vi "Guardian Died Recheck.vi"(8 "error in (no error)":errorcluster, 10 "ID":string, 11 "Guardian in":refnum<class "Guardian.lvclass">) -> (0 "error out":errorcluster, 3 "Guardian out":refnum<class "Guardian.lvclass">)   [LabVIEW 2020, in "TALOS.lvlib" / "Guardian.lvlib" / "Guardian.lvclass"]
doc: "This VI gets scheduled to be run whenever a Guardian is found to be not updating its Guardian_Health ASV: if the Guardian is found alive, nothing is done, while if it is really found dead, ABORT is raised."
uses:
  Guardian.lvclass
  Guardian.lvclass/Guardian.ctl
  TALOS.lvlib
  Classes/Distributed uService Map/Distributed uService Map.lvclass
  d99af1e7-28a1-4e92-bcbf-3239d693d740.vi
  Ancestor/Ancestor/Ancestor.lvclass
  C:/LabVIEW Code/TALOS/talos/Ancestor/Ancestor/Ancestor.lvclass
  C:/LabVIEW Code/TALOS/builds/Actor Framework PPL/Actor Framework.lvlibp/1abvi3w/vi.lib/ActorFramework/Actor/Actor.lvclass
  C:/LabVIEW Code/TALOS/talos/Guardian/Guardian/Guardian.lvclass
  Classes/Guardian List/Guardian List.lvclass
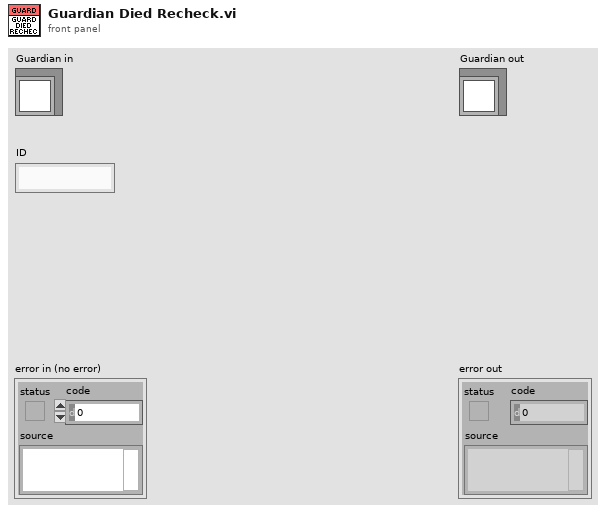
[diagram p1: front panel]
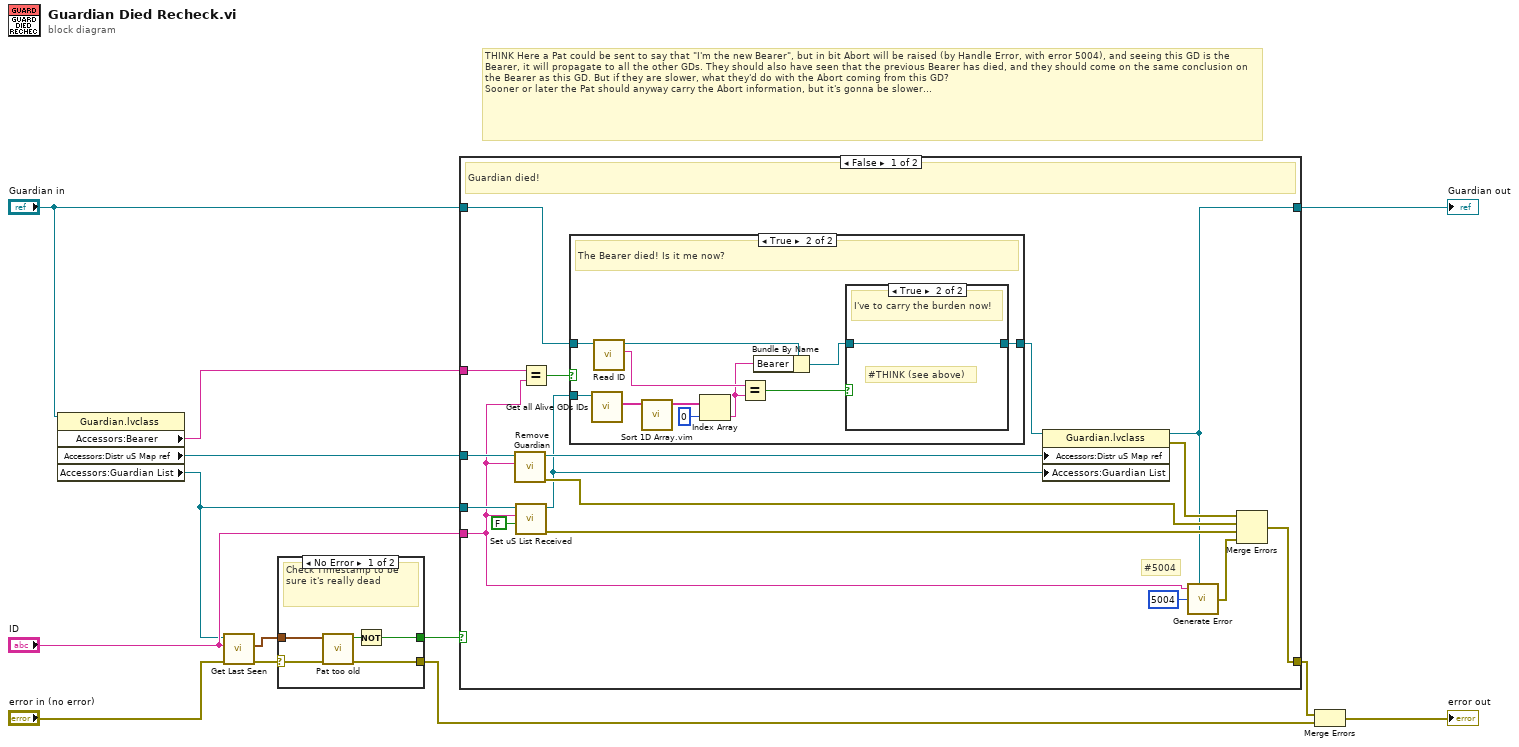
[diagram p0: block diagram]
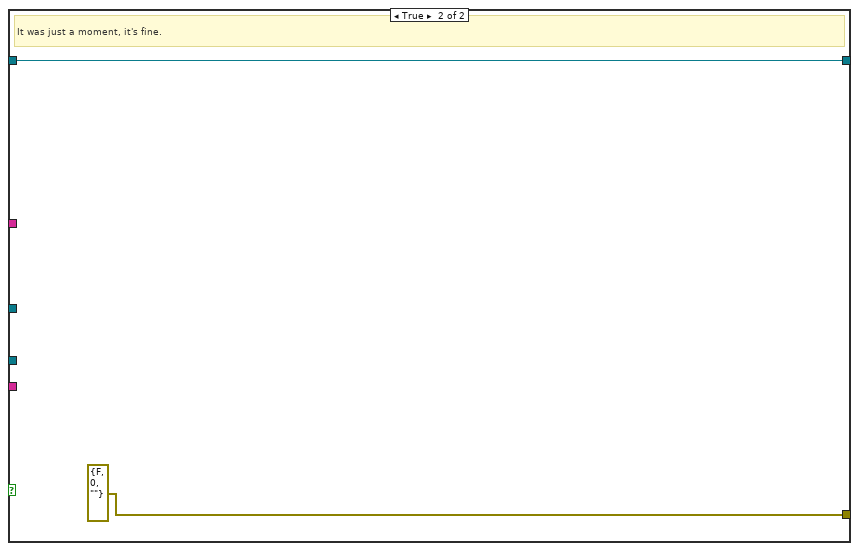
[diagram p4: hidden frame]
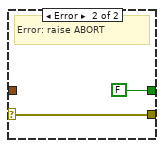
[diagram p5: hidden frame]
diagram:
  # "THINK Here a Pat could be sent to say that \"I'm the new Bearer\", but in bit Abort will be raised (by Handle Error, with error 5004), and seeing this GD is the Bearer, it will propagate to all the other GDs. They should also have seen that the previous Bearer has died, and they should come on the same conclusion on the Bearer as this GD. But if they are slower, what they'd do with the Abort coming from this GD? \nSooner or later the Pat should anyway carry the Abort information, but it's gonna be slower..."
  n1 = property class="Guardian.lvclass"(reference="Guardian in") -> ("Accessors:Bearer"=w1:string, "Accessors:Distr uS Map ref"=w2:refnum<data-value>, "Accessors:Guardian List"=w3:refnum<class "Guardian List.lvclass">)  [unwired: 1 in, 2 out]
  n2 = call-dynamic "Get Last Seen.vi"("error in (no error)"="error in (no error)", "ID"="ID", "Guardian List in"=w3) -> ("error out"=w8:errorcluster, "Last Poke"=w9:timestamp)  [unwired: 6 in, 1 out]
  n3 = case shown="No Error" w8 {
    selector: w8 -> [w15 w19]
    tunnel: w9 -> [w18 _]
    tunnel: [w16 FALSE] -> w11
    tunnel: [w14 w19] -> w7
    frame No Error {
      # "Check Timestamp to be sure it's really dead"
      n4 = call "Pat too old.vi"("error in (no error)"=w15, "Last Seen"=w18) -> ("error out"=w14:errorcluster, "Too old?"=w17:bool)  [unwired: 8 in]
      n5 = Not(x=w17) -> (.not. x?=w16:bool)
    }
    frame Error {
      # "Error: raise ABORT"
    }
  }
  n6 = case shown="False" w11 {
    tunnel: [w34 errorcluster {"status"=FALSE, "code"=0, "source"=""} ("error out")] -> w12
    tunnel: "Guardian in" -> [w26 w52]
    tunnel: w3 -> [w33 _]
    tunnel: "ID" -> [w28 _]
    tunnel: [w22 w52] -> w5
    tunnel: w2 -> [w30 _]
    tunnel: w1 -> [w21 _]
    frame False {
      # "#5004"
      # "Guardian died!"
      n7 = call "Remove Guardian.vi"("Guardian ID"=w28, "Distr uS Map ref in"=w30) -> ("error out"=w29:errorcluster, "Distr uS Map ref out"=w24:refnum<data-value>)  [unwired: 8 in]
      n8 = call-dynamic "Set uS List Received.vi"("uS List Received"=FALSE, "ID"=w28, "Guardian List in"=w33) -> ("error out"=w31:errorcluster, "Guardian List out"=w23:refnum<class "Guardian List.lvclass">)  [unwired: 7 in]
      n9 = Equal?(x=w21, y=w28) -> (x = y?=w27:bool)
      n10 = case shown="True" w27 {
        tunnel: w23 -> [_ w49]
        tunnel: w26 -> [w38 w45]
        tunnel: [w38 w39] -> w25
        frame False {
          # "The dead GD was not the Bearer, all good."
        }
        frame True {
          # "The Bearer died! Is it me now?"
          n11 = call-dynamic "Get all Alive GDs IDs.vi"("Guardian List in"=w49) -> ("Alive GDs IDs"=w48:string[])  [unwired: 8 in, 2 out]
          n12 = call "Read ID.vi"("Ancestor in"=w45) -> ("ID"=w42:string, "Ancestor out"=w43:refnum<class "Guardian.lvclass">)  [unwired: 8 in, 1 out]
          n13 = call "Sort 1D Array.vim"("unsorted array"=w48) -> ("sorted array"=w47:string[])  [unwired: 10 in]
          n14 = Index Array(array=w47, index=0) -> (element=w41:string)
          n15 = Equal?(x=w42, y=w41) -> (x = y?=w44:bool)
          n16 = Bundle By Name(cluster=w43, "Bearer"=w41) -> (w40:refnum<class "Guardian.lvclass">)
          n17 = case shown="True" w44 {
            tunnel: w40 -> [w50 w51]
            tunnel: [w50 w51] -> w39
            frame False {
              # "No (do nothing)"
            }
            frame True {
              # "#THINK (see above)"
              # "I've to carry the burden now!"
            }
          }
        }
      }
      n18 = property class="Guardian.lvclass"(reference=w25, "Accessors:Distr uS Map ref"=w24, "Accessors:Guardian List"=w23) -> (reference out=w22:refnum<class "Guardian.lvclass">, error out=w37:errorcluster)  [unwired: 1 in]
      n19 = call "Generate Error.vi"("Optional String"=w28, "Class"=w22, "Error Code"=5004) -> ("error out"=w35:errorcluster)  [unwired: 4 in]
      n20 = Merge Errors(w37, w29, w31, w35) -> (w34:errorcluster)
    }
    frame True {
      # "It was just a moment, it's fine."
    }
  }
  "Guardian out" <- w5
  n21 = Merge Errors(w12, w7) -> (→"error out":errorcluster)
